vi "Get Control Reference.vi"(8 "error in":errorcluster, 11 "Element in":refnum<class "Element.lvclass">) -> (0 "error out":errorcluster, 2 "Control Reference":refnum<vi>, 3 "Element out":refnum<class "Element.lvclass">)   [LabVIEW 2026, in "Element.lvclass"]
doc: "Get Control Reference."
uses:
  Element.lvclass
  Element.lvclass/Element.ctl
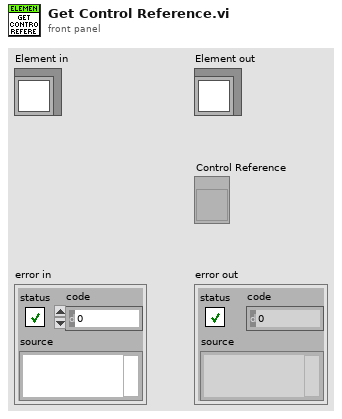
[diagram p1: front panel]
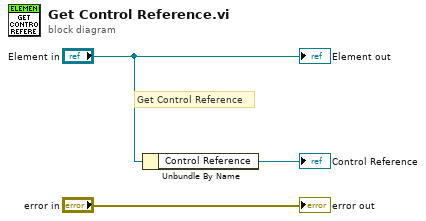
[diagram p0: block diagram]
diagram:
  # "Get Control Reference"
  n1 = Unbundle By Name("Element in") -> ("Control Reference"=→"Control Reference":refnum<vi>)
  "error out" <- "error in"
  "Element out" <- "Element in"
